vi "init Sweep Measurement.vi"(8 "error in (no error)":errorcluster, 10 "Sweep Measurement Mode":enum16{"Single Sweep", "Continuous Sweep"}(ring), 11 "Keysight 9020A in":refnum<class "Keysight 9020A.lvclass">) -> (0 "error out":errorcluster, 3 "Keysight 9020A out":refnum<class "Keysight 9020A.lvclass">)   [LabVIEW 2023, in "Spectrum Analyzer.lvlib" / "Keysight 9020A.lvclass"]
uses:
  Keysight 9020A.lvclass
  Keysight 9020A.lvclass/Keysight 9020A.ctl
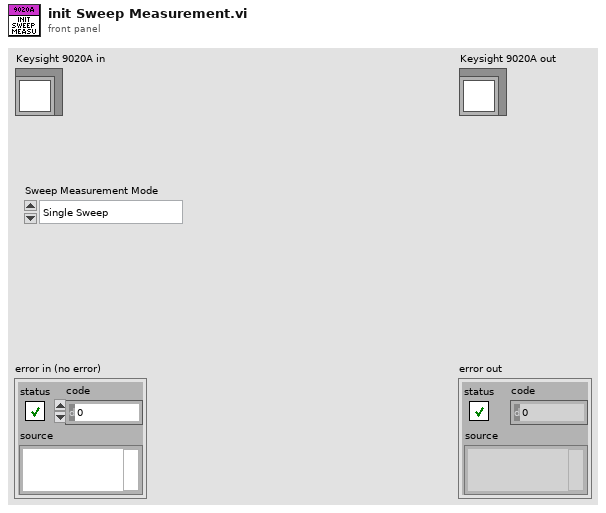
[diagram p1: front panel]
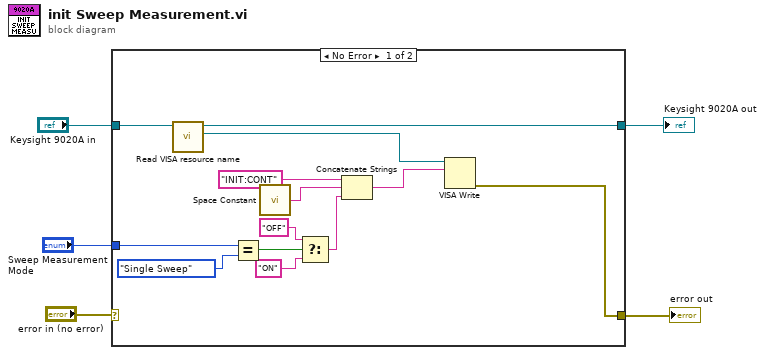
[diagram p0: block diagram]
diagram:
  n1 = case shown="No Error" "error in (no error)" {
    selector: "error in (no error)" -> [_ w20]
    tunnel: "Keysight 9020A in" -> [w8 w19]
    tunnel: [w9 w20] -> w1
    tunnel: [w7 w19] -> w4
    tunnel: "Sweep Measurement Mode" -> [w16 _]
    frame No Error {
      n2 = call "Read VISA resource name.vi"("Keysight 9020A in"=w8) -> ("VISA resource name"=w6:refnum<visa-resource-name>, "Keysight 9020A out"=w7:refnum<class "Keysight 9020A.lvclass">)  [unwired: 8 in, 1 out]
      n3 = Equal?(x=w16, y=enum16{"Single Sweep", "Continuous Sweep"}."Single Sweep") -> (x = y?=w14:bool)
      n4 = call <vilib>:"Space Constant.vi"() -> ("String"=w17:string)
      n5 = Select(t="OFF", s=w14, f="ON") -> (s? t:f=w11:string)
      n6 = Concatenate Strings("INIT:CONT" ("string"), w17, w11) -> (w10:string)
      n7 = VISA Write(VISA resource name=w6, write buffer=w10) -> (error out=w9:errorcluster)  [unwired: 1 in, 2 out]
    }
    frame Error {
    }
  }
  "error out" <- w1
  "Keysight 9020A out" <- w4
